vi "Read Numeric Channel Properties.vi"(7 "Input?":bool, 8 "error in (no error)":errorcluster, 10 "Numeric Channel ID":string, 11 "Channel in":refnum<class "Channel.lvclass">) -> (0 "error out":errorcluster, 2 "Numeric Channel":T1, 3 "Channel out":refnum<class "Channel.lvclass">)   [LabVIEW 2026, in "Modbus.lvlib" / "Modbus.lvclass"]
uses:
  Modbus.lvclass
  <vilib>/FlexLogger/SDK/PluginSDK.lvlibp/PEFClasses/SDK/Channel/Channel.lvclass
  Types/Numeric Data.ctl
  Types/Modbus Table.ctl
  Types/Numeric Size.ctl
  Types/Numeric Data Type.ctl
  Types/Numeric Location.ctl
  Globals/Modbus Strings.vi
  <vilib>/FlexLogger/SDK/PluginSDK.lvlibp/PEFClasses/SDK/Channel/ParameterAccess/Read Enum.vi
  <vilib>/FlexLogger/SDK/PluginSDK.lvlibp/PEFClasses/SDK/Channel/ParameterAccess/Read I32.vi
  <vilib>/FlexLogger/SDK/PluginSDK.lvlibp/PEFClasses/SDK/Channel/Read Valid.vi
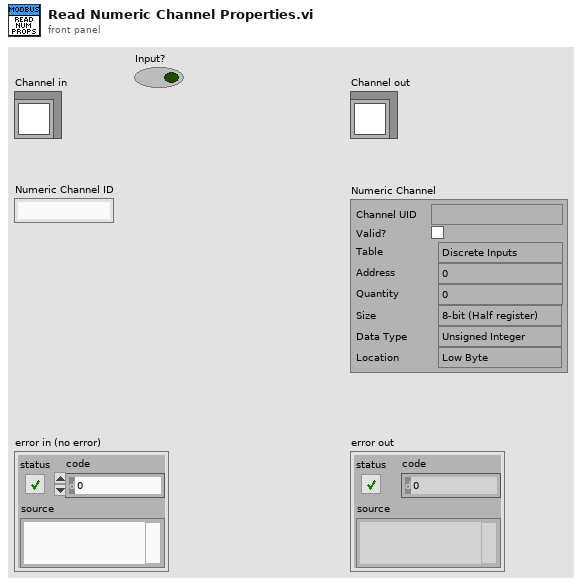
[diagram p1: front panel]
types:
  T1 = typedef "Modbus.lvlib/Modbus.lvclass/Numeric Data.ctl" = cluster{"Channel UID":string, "Valid?":bool, "Table":T2, "Address":i32, "Quantity":u16, "Size":T3, "Data Type":T4, "Location":T5}
  T2 = typedef "Modbus.lvlib/Modbus.lvclass/Modbus Table.ctl" = enum16{"Discrete Inputs", "Coils", "Input Registers", "Holding Registers"}
  T3 = typedef "Modbus.lvlib/Modbus.lvclass/Numeric Size.ctl" = enum16{"8-bit (Half register)", "16-bit (One register)", "32-bit (Two registers)", "64-bit (Four registers)"}
  T4 = typedef "Modbus.lvlib/Modbus.lvclass/Numeric Data Type.ctl" = enum16{"Unsigned Integer", "Signed Integer", "Floating Point"}
  T5 = typedef "Modbus.lvlib/Modbus.lvclass/Numeric Location.ctl" = enum16{"Low Byte", "High Byte"}
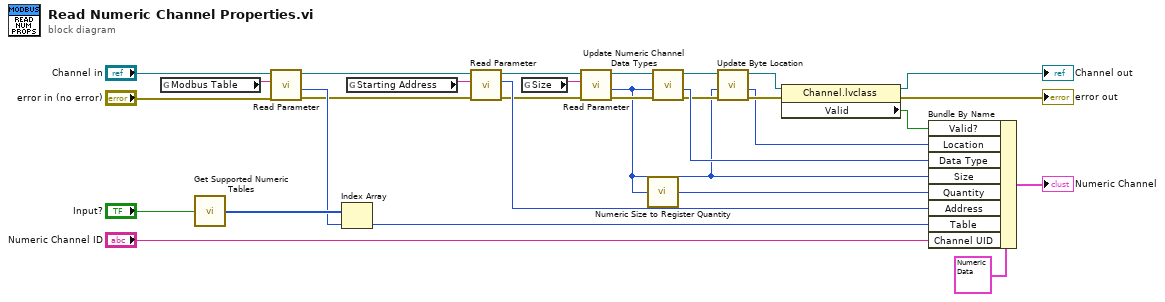
[diagram p0: block diagram]
diagram:
  n1 = global read "Modbus Strings.vi" "Modbus Table"() -> (w22:string)
  n2 = call "Get Supported Numeric Tables.vi"("Input?"="Input?") -> ("Supported Tables"=w30:T2[])
  n3 = call-poly <vilib>:"Read Parameter.vi"("error in (no error)"="error in (no error)", "Name"=w22, "Channel in"="Channel in") -> ("error out"=w24:errorcluster, "Index"=w26:i32, "Channel out"=w23:refnum<class "Channel.lvclass">)  [unwired: 4 in, 2 out]
  n4 = Index Array(array=w30, index=w26) -> (element=w27:T2)
  n5 = global read "Modbus Strings.vi" "Starting Address"() -> (w25:string)
  n6 = call-poly <vilib>:"Read Parameter.vi"("error in (no error)"=w24, "Name"=w25, "Channel in"=w23) -> ("error out"=w12:errorcluster, "Value"=w28:i32, "Channel out"=w13:refnum<class "Channel.lvclass">)  [unwired: 5 in, 1 out]
  n7 = global read "Modbus Strings.vi" "Size"() -> (w11:string)
  n8 = call-poly <vilib>:"Read Parameter.vi"("error in (no error)"=w12, "Name"=w11, "Channel in"=w13) -> ("error out"=w8:errorcluster, "Index"=w2:i32, "Channel out"=w9:refnum<class "Channel.lvclass">)  [unwired: 4 in, 2 out]
  n9 = call "Numeric Size to Register Quantity.vi"("Size"=w2) -> ("Quantity"=w10:u16)
  n10 = call "Update Numeric Channel Data Types.vi"("error in (no error)"=w8, "Size"=w2, "Channel in"=w9) -> ("error out"=w5:errorcluster, "Selected Data Type"=w7:T4, "Channel out"=w6:refnum<class "Channel.lvclass">)  [unwired: 6 in]
  n11 = call "Update Byte Location.vi"("error in (no error)"=w5, "Size"=w2, "Channel in"=w6) -> ("error out"=w4:errorcluster, "Location"=w1:T5, "Channel out"=w3:refnum<class "Channel.lvclass">)  [unwired: 6 in]
  n12 = property class="Channel.lvclass"(reference=w3, error in=w4) -> (reference out=→"Channel out":refnum<class "Channel.lvclass">, error out=→"error out":errorcluster, "Valid"=w17:bool)
  n13 = Bundle By Name(cluster=T1 {"Channel UID"="", "Valid?"=FALSE, "Table"=enum."Discrete Inputs", "Address"=0, "Quantity"=0, "Size"=enum."8-bit (Half register)", "Data Type"=enum."Unsigned Integer", "Location"=enum."Low Byte"} ("Numeric Data"), "Valid?"=w17, "Location"=w1, "Data Type"=w7, "Size"=w2, "Quantity"=w10, "Address"=w28, "Table"=w27, "Channel UID"="Numeric Channel ID") -> (→"Numeric Channel":T1)
